vi "Move_Air.vi"(0 "State":T1={"Tick"=0, "Phase"=0, "PhaseTicks"=0, "Level"=1, "Room"=0, "X10"=0, "Y10"=0, "VY10"=0, "Mode"=0, "Facing"=0, "Run"=0, "Vert"=0, "StandY"=0, "EntryX10"=0, "EntryY10"=0, "EntryMode"=0, "Lives"=4, "Score"=0, "NextLife"=10000, "KeyR"=0, "KeyB"=0, "KeyY"=0, "Torch"=FALSE, "FloorPhase"=0, "Dead"=FALSE, "LevelStart"=FALSE, "Quit"=FALSE, "Sound"=0, "Seed"=12345, "DemoStep"=0, "Tiles"=[], "World"=[], "Enemies"=[], "Highscores"=[], "Name"=[0, 0, 0], "Cursor"=0}, 7 "XA10":i32, 11 "error in":errorcluster) -> (4 "Mode":i32, 6 "X10":i32, 8 "Y10":i32, 10 "VY10":i32, 13 "Dead":bool, 15 "error out":errorcluster)   [LabVIEW 2020, in "GH_Engine.lvlib"]
doc: "Claude in the air, one tick: gravity (parachute in the treasure room), head bump, landing on walls, thin floors (only from above) and ladder tops, grabbing a ladder (with Up/Down), a rope or a pole while falling. Dead = landed more than the allowed height below the last firm stand (never with the parachute). Inline subVI of Player_Move."
uses:
  GH_Engine.lvlib
  Level/GH_Level.lvlib
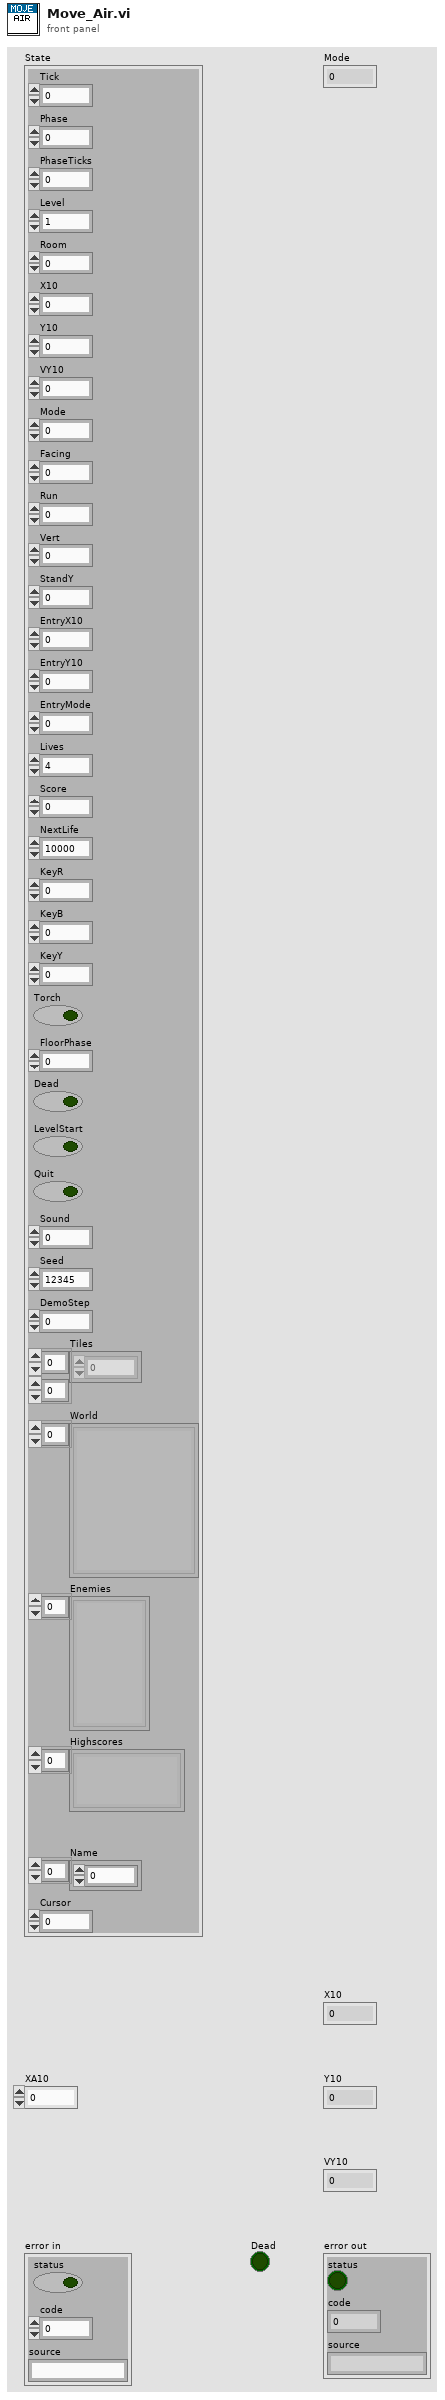
[diagram p1: front panel]
types:
  T1 = cluster{"Tick":u32, "Phase":i32, "PhaseTicks":i32, "Level":i32, "Room":i32, "X10":i32, "Y10":i32, "VY10":i32, "Mode":i32, "Facing":i32, "Run":i32, "Vert":i32, "StandY":i32, "EntryX10":i32, "EntryY10":i32, "EntryMode":i32, "Lives":i32, "Score":i32, "NextLife":i32, "KeyR":i32, "KeyB":i32, "KeyY":i32, "Torch":bool, "FloorPhase":i32, "Dead":bool, "LevelStart":bool, "Quit":bool, "Sound":i32, "Seed":u32, "DemoStep":i32, "Tiles":u8[][], "World":cluster{"ID":string, "Depth":i32, "Column":i32, "Tiles":u8[][]}[], "Enemies":cluster{"Kind":i32, "X10":i32, "Y10":i32, "Dir":i32, "Mode":i32}[], "Highscores":cluster{"Score":i32, "Name":string}[], "Name":i32[], "Cursor":i32}
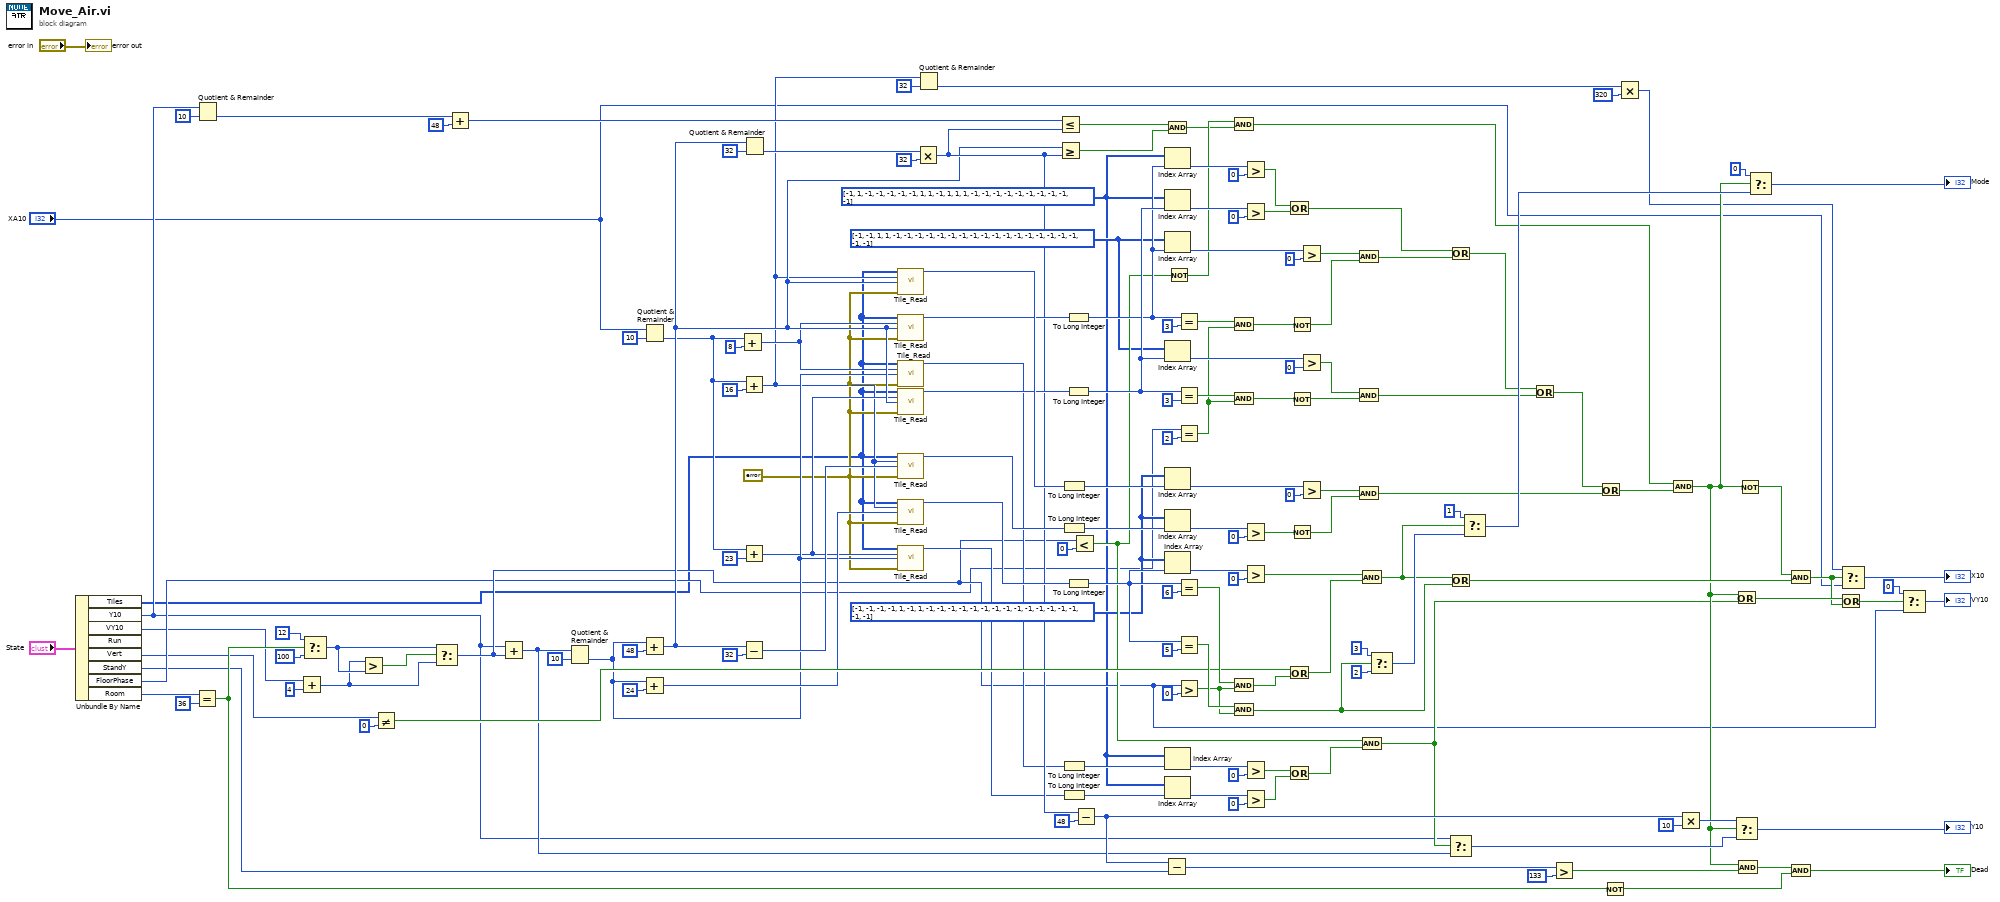
[diagram p0: block diagram]
diagram:
  w16 = errorcluster {"status"=FALSE, "code"=0, "source"=""} ("no error")
  w13 = i32[] [-1, -1, -1, -1, 1, -1, 1, -1, -1, -1, -1, -1, -1, -1, -1, -1, -1, -1, -1, -1, -1, -1, -1] ("Ladder or rope")
  w12 = i32[] [-1, -1, 1, 1, -1, -1, -1, -1, -1, -1, -1, -1, -1, -1, -1, -1, -1, -1, -1, -1, -1, -1, -1] ("Thin floor")
  w11 = i32[] [-1, 1, -1, -1, -1, -1, -1, 1, 1, -1, 1, 1, 1, -1, -1, -1, -1, -1, -1, -1, -1, -1, -1] ("Solid")
  n1 = Unbundle By Name("State") -> ("Tiles"=w4:u8[][], "Y10"=w5:i32, "VY10"=w6:i32, "Vert"=w7:i32, "StandY"=w8:i32, "FloorPhase"=w9:i32, "Room"=w10:i32)  [unwired: 1 out]
  n2 = Equal?(x=w10, y=36) -> (x = y?=w34:bool)
  n3 = Quotient & Remainder(x=w5, y=10) -> (floor(x/y)=w26:i32)  [unwired: 1 out]
  n4 = Add(x=w6, y=4) -> (x+y=w36:i32)
  n5 = Select(t=12, s=w34, f=100) -> (s? t:f=w39:i32)
  n6 = Greater?(x=w36, y=w39) -> (0:w40:bool)
  n7 = Not Equal?(x=w7, y=0) -> (x != y?=w127:bool)
  n8 = Select(t=w39, s=w40, f=w36) -> (s? t:f=w41:i32)
  n9 = Add(x=w26, y=48) -> (x+y=w28:i32)
  n10 = Add(x=w5, y=w41) -> (x+y=w42:i32)
  n11 = Quotient & Remainder(x=w42, y=10) -> (floor(x/y)=w44:i32)  [unwired: 1 out]
  n12 = Add(x=w44, y=48) -> (x+y=w46:i32)
  n13 = Add(x=w44, y=24) -> (x+y=w118:i32)
  n14 = Quotient & Remainder(x="XA10", y=10) -> (floor(x/y)=w18:i32)  [unwired: 1 out]
  n15 = Add(x=w18, y=8) -> (x+y=w22:i32)
  n16 = Add(x=w18, y=16) -> (x+y=w20:i32)
  n17 = Add(x=w18, y=23) -> (x+y=w24:i32)
  n18 = Subtract(x=w46, y=32) -> (x-y=w78:i32)
  n19 = Quotient & Remainder(x=w46, y=32) -> (floor(x/y)=w62:i32)  [unwired: 1 out]
  n20 = call "Tile_Read.vi"("Tiles"=w4, "X"=w20, "Y"=w46, "error in"=w16) -> ("Tile"=w72:u8)  [unwired: 10 in, 1 out]
  n21 = call "Tile_Read.vi"("Tiles"=w4, "X"=w22, "Y"=w46, "error in"=w16) -> ("Tile"=w68:u8)  [unwired: 10 in, 1 out]
  n22 = call "Tile_Read.vi"("Tiles"=w4, "X"=w22, "Y"=w44, "error in"=w16) -> ("Tile"=w49:u8)  [unwired: 10 in, 1 out]
  n23 = call "Tile_Read.vi"("Tiles"=w4, "X"=w24, "Y"=w46, "error in"=w16) -> ("Tile"=w70:u8)  [unwired: 10 in, 1 out]
  n24 = call "Tile_Read.vi"("Tiles"=w4, "X"=w20, "Y"=w78, "error in"=w16) -> ("Tile"=w79:u8)  [unwired: 10 in, 1 out]
  n25 = call "Tile_Read.vi"("Tiles"=w4, "X"=w20, "Y"=w118, "error in"=w16) -> ("Tile"=w119:u8)  [unwired: 10 in, 1 out]
  n26 = call "Tile_Read.vi"("Tiles"=w4, "X"=w24, "Y"=w44, "error in"=w16) -> ("Tile"=w54:u8)  [unwired: 10 in, 1 out]
  n27 = Multiply(x=w62, y=32) -> (x*y=w64:i32)
  n28 = Quotient & Remainder(x=w20, y=32) -> (floor(x/y)=w30:i32)  [unwired: 1 out]
  n29 = Less Or Equal?(x=w28, y=w64) -> (x <= y?=w65:bool)
  n30 = Greater Or Equal?(x=w46, y=w64) -> (x >= y?=w66:bool)
  n31 = To Long Integer(number=w72) -> (32bit integer=w73:i32)
  n32 = To Long Integer(number=w79) -> (32bit integer=w80:i32)
  n33 = To Long Integer(number=w49) -> (32bit integer=w50:i32)
  n34 = To Long Integer(number=w54) -> (32bit integer=w55:i32)
  n35 = To Long Integer(number=w68) -> (32bit integer=w69:i32)
  n36 = To Long Integer(number=w70) -> (32bit integer=w71:i32)
  n37 = To Long Integer(number=w119) -> (32bit integer=w120:i32)
  n38 = Less?(x=w41, y=0) -> (x < y?=w48:bool)
  n39 = Subtract(x=w64, y=48) -> (x-y=w116:i32)
  n40 = Subtract(x=w116, y=w8) -> (x-y=w155:i32)
  n41 = And(x=w65, y=w66) -> (x .and. y?=w67:bool)
  n42 = Index Array(array=w11, index=w69) -> (element=w87:i32)
  n43 = Index Array(array=w11, index=w71) -> (element=w90:i32)
  n44 = Index Array(array=w12, index=w69) -> (element=w93:i32)
  n45 = Index Array(array=w12, index=w71) -> (element=w101:i32)
  n46 = Index Array(array=w13, index=w73) -> (element=w74:i32)
  n47 = Index Array(array=w13, index=w80) -> (element=w81:i32)
  n48 = Index Array(array=w13, index=w120) -> (element=w123:i32)
  n49 = Index Array(array=w11, index=w50) -> (element=w51:i32)
  n50 = Index Array(array=w11, index=w55) -> (element=w56:i32)
  n51 = Not(x=w48) -> (.not. x?=w86:bool)
  n52 = Equal?(x=w69, y=3) -> (x = y?=w97:bool)
  n53 = Equal?(x=w71, y=3) -> (x = y?=w105:bool)
  n54 = Equal?(x=w9, y=2) -> (x = y?=w15:bool)
  n55 = Equal?(x=w120, y=6) -> (x = y?=w129:bool)
  n56 = Equal?(x=w120, y=5) -> (x = y?=w134:bool)
  n57 = Greater?(x=w41, y=0) -> (0:w122:bool)
  n58 = And(x=w86, y=w67) -> (x .and. y?=w113:bool)
  n59 = And(x=w97, y=w15) -> (x .and. y?=w98:bool)
  n60 = And(x=w105, y=w15) -> (x .and. y?=w106:bool)
  n61 = And(x=w129, y=w122) -> (x .and. y?=w130:bool)
  n62 = And(x=w134, y=w122) -> (x .and. y?=w135:bool)
  n63 = Greater?(x=w87, y=0) -> (0:w89:bool)
  n64 = Greater?(x=w90, y=0) -> (0:w92:bool)
  n65 = Greater?(x=w81, y=0) -> (0:w83:bool)
  n66 = Greater?(x=w123, y=0) -> (0:w125:bool)
  n67 = Greater?(x=w51, y=0) -> (0:w53:bool)
  n68 = Greater?(x=w56, y=0) -> (0:w58:bool)
  n69 = Or(x=w89, y=w92) -> (x .or. y?=w109:bool)
  n70 = Or(x=w127, y=w130) -> (x .or. y?=w131:bool)
  n71 = Or(x=w53, y=w58) -> (x .or. y?=w59:bool)
  n72 = Not(x=w98) -> (.not. x?=w99:bool)
  n73 = Not(x=w106) -> (.not. x?=w107:bool)
  n74 = Not(x=w83) -> (.not. x?=w84:bool)
  n75 = Greater?(x=w93, y=0) -> (0:w95:bool)
  n76 = Greater?(x=w101, y=0) -> (0:w103:bool)
  n77 = Greater?(x=w74, y=0) -> (0:w76:bool)
  n78 = And(x=w95, y=w99) -> (x .and. y?=w100:bool)
  n79 = And(x=w103, y=w107) -> (x .and. y?=w108:bool)
  n80 = And(x=w76, y=w84) -> (x .and. y?=w85:bool)
  n81 = And(x=w125, y=w131) -> (x .and. y?=w132:bool)
  n82 = And(x=w48, y=w59) -> (x .and. y?=w60:bool)
  n83 = Select(t=3, s=w135, f=2) -> (s? t:f=w143:i32)
  n84 = Or(x=w109, y=w100) -> (x .or. y?=w110:bool)
  n85 = Or(x=w132, y=w135) -> (x .or. y?=w137:bool)
  n86 = Select(t=w5, s=w60, f=w42) -> (s? t:f=w149:i32)
  n87 = Select(t=1, s=w132, f=w143) -> (s? t:f=w144:i32)
  n88 = Or(x=w110, y=w108) -> (x .or. y?=w111:bool)
  n89 = Greater?(x=w155, y=133) -> (0:w157:bool)
  n90 = Or(x=w111, y=w85) -> (x .or. y?=w112:bool)
  n91 = Not(x=w34) -> (.not. x?=w158:bool)
  n92 = Multiply(x=w30, y=320) -> (x*y=w32:i32)
  n93 = And(x=w113, y=w112) -> (x .and. y?=w114:bool)
  n94 = Multiply(x=w116, y=10) -> (x*y=w148:i32)
  n95 = Or(x=w114, y=w60) -> (x .or. y?=w151:bool)
  n96 = Select(t=w148, s=w114, f=w149) -> (s? t:f=→"Y10":i32)
  n97 = And(x=w114, y=w157) -> (x .and. y?=w159:bool)
  n98 = Not(x=w114) -> (.not. x?=w136:bool)
  n99 = Select(t=0, s=w114, f=w144) -> (s? t:f=→"Mode":i32)
  n100 = And(x=w136, y=w137) -> (x .and. y?=w138:bool)
  n101 = And(x=w159, y=w158) -> (x .and. y?=→"Dead":bool)
  n102 = Or(x=w151, y=w138) -> (x .or. y?=w152:bool)
  n103 = Select(t=w32, s=w138, f="XA10") -> (s? t:f=→"X10":i32)
  n104 = Select(t=0, s=w152, f=w41) -> (s? t:f=→"VY10":i32)
  "error out" <- "error in"
